vi "monitoring_center.vi"() -> ()   [LabVIEW 2026]
panel:
  out "Array":cluster{i32[], "p":dbl[]}[](array[cluster])
  out "XY Graph":cluster{i32[], "p":dbl[]}[](graph)
  in  "Nodes":T1(array[cluster])
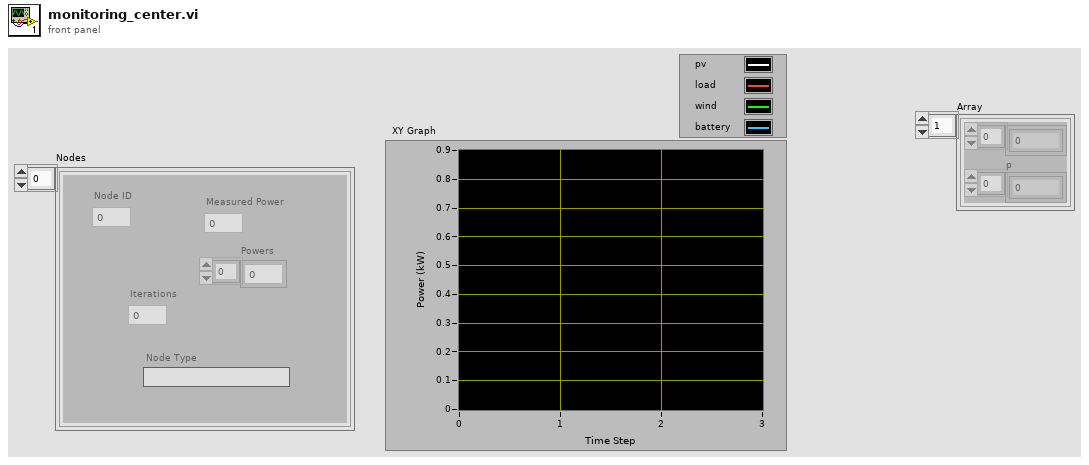
[diagram p1: front panel]
types:
  T1 = cluster{"node_id":i32, "measured_power":dbl, "iterations":i32, "node_type":string, "p":dbl[]}[]
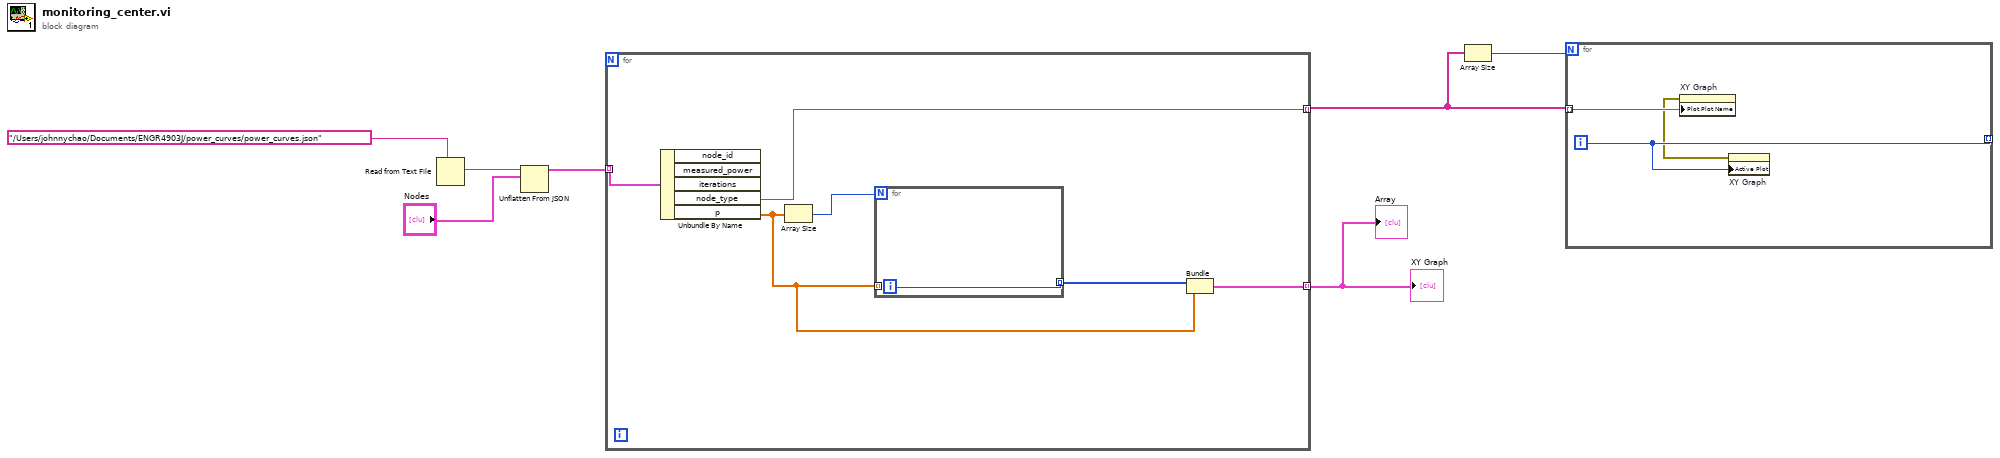
[diagram p0: block diagram]
diagram:
  n1 = Read from Text File(prompt (Open existing file)="/Users/johnnychao/Documents/ENGR4903J/power_curves/power_curves.json") -> (text=w6:string)  [unwired: 3 in, 3 out]
  n2 = Unflatten From JSON(JSON string=w6, type and defaults="Nodes") -> (value=w4:T1)  [unwired: 5 in, 1 out]
  n3 = for {
    tunnel: w4 -> [w13] mode=indexing
    tunnel: [w10] -> w3 mode=indexing
    tunnel: [w8] -> w1 mode=indexing
    n4 = Unbundle By Name(w13) -> ("node_type"=w8:string, "p"=w9:dbl[])  [unwired: 3 out]
    n5 = Array Size(array=w9) -> (size(s)=w12:i32)
    n6 = for {
      N: w12 -> [_]
      tunnel: w9 -> [_] mode=indexing
      tunnel: [w14] -> w11 mode=indexing
      i -> [w14]
    }
    n7 = Bundle(w11, "p"=w9) -> (w10:cluster{i32[], "p":dbl[]})  [unwired: 1 in]
  }
  "XY Graph" <- w3
  "Array" <- w3
  n8 = Array Size(array=w1) -> (size(s)=w2:i32)
  n9 = for {
    N: w2 -> [_]
    tunnel: [w16] -> _ mode=indexing
    tunnel: w1 -> [w17] mode=indexing
    i -> [w16]
    n10 = property on="XY Graph" class="XYGraph (strict)"("Active Plot"=w16) -> (error out=w15:errorcluster)  [unwired: 2 in, 1 out]
    n11 = property on="XY Graph" class="XYGraph (strict)"(error in=w15, "Plot.Plot Name"=w17) -> ()  [unwired: 1 in, 2 out]
  }
